vi "RemoteVI Copy Text.vi"(0 "text":string) -> (15 "error out":errorcluster)   [LabVIEW 2020, in "RemoteVI.lvlib"]
doc: "Puts text on the Windows clipboard (clip.exe reads it from standard input, through System Exec.vi). RemoteVI Server's Copy link."
uses:
  RemoteVI.lvlib
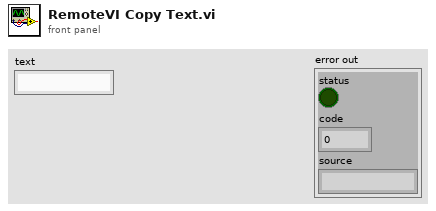
[diagram p1: front panel]
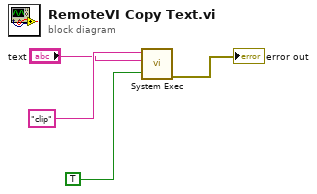
[diagram p0: block diagram]
diagram:
  n1 = call <vilib>:"System Exec.vi"("run minimized? (F)"=TRUE, "standard input"="text", "command line"="clip") -> ("error out"=→"error out":errorcluster)  [unwired: 5 in, 3 out]
